vi "PackData.vi"(10 "字符串输入":string, 11 "Data Type":T1) -> (3 "字符串输出":string)   [LabVIEW 2020, in "TCP Communication.lvlib"]
uses:
  TCP Communication.lvlib
  Data Type.ctl
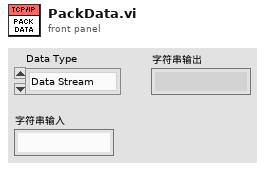
[diagram p1: front panel]
types:
  T1 = typedef "TCP Communication.lvlib/Data Type.ctl" = enum16{"Data Stream", "Status", "Request", "Reply"}
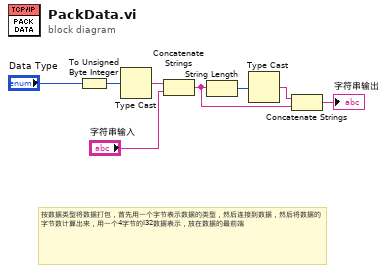
[diagram p0: block diagram]
diagram:
  # "按数据类型将数据打包，首先用一个字节表示数据的类型，然后连接到数据，然后将数据的字节数计算出来，用一个4字节的I32数据表示，放在数据的最前端"
  n1 = To Unsigned Byte Integer(number="Data Type") -> (unsigned 8bit integer=w8:u8)
  n2 = Type Cast(x=w8) -> (*(type *) &x=w2:string)  [unwired: 1 in]
  n3 = Concatenate Strings(w2, "字符串输入") -> (w3:string)
  n4 = String Length(string=w3) -> (length=w5:i32)
  n5 = Type Cast(x=w5) -> (*(type *) &x=w4:string)  [unwired: 1 in]
  n6 = Concatenate Strings(w4, w3) -> (→"字符串输出":string)
